vi "shear_and_recovery_integral_calculation__45bec310ce.vi"(7 "frequency":dbl, 8 "amplitude":dbl=1.0 format="%0.2f", 9 "loop period (ms)":dbl, 10 "recovery phase (half period=32)":dbl, 11 "# periods":i32) -> ()   [LabVIEW 2023]
uses:
  <vilib>/Analysis/NI_AALBase.lvlib
panel:
  out "Waveform Graph":dbl[](graph)
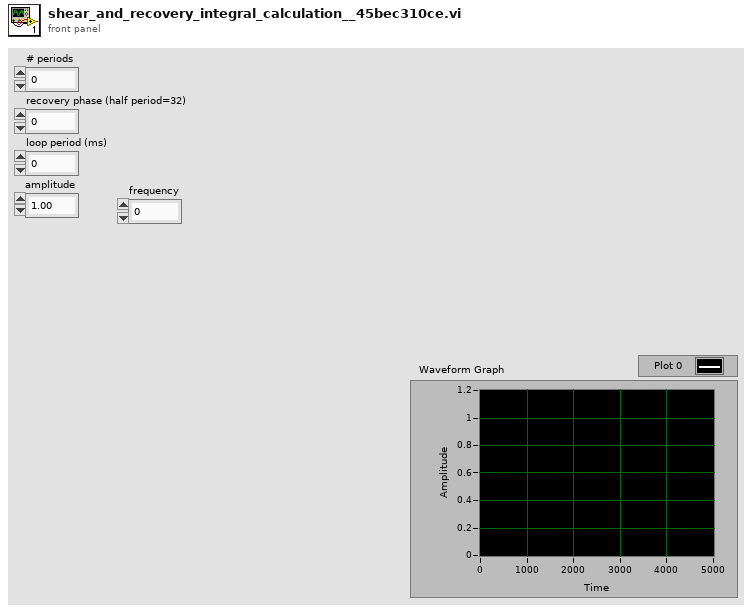
[diagram p1: front panel]
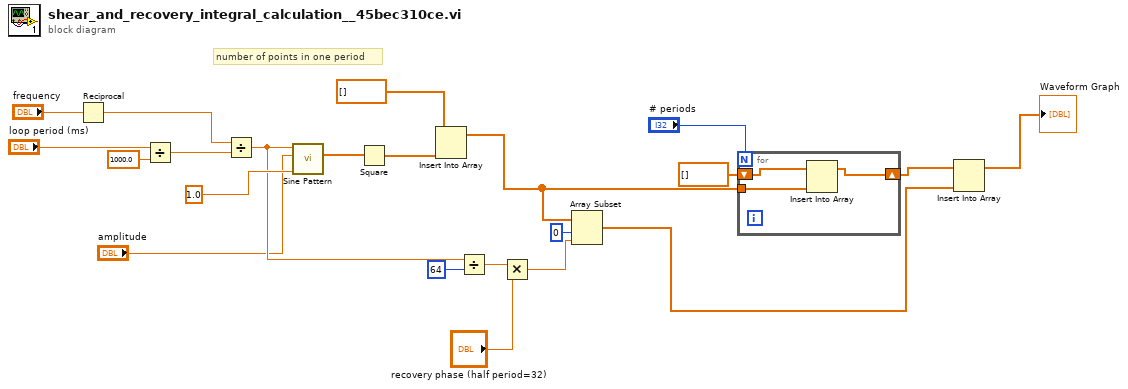
[diagram p0: block diagram]
diagram:
  # "number of points in one period"
  n1 = Reciprocal(x="frequency") -> (1/x=w8:dbl)
  n2 = Divide(x="loop period (ms)", y=1000.0) -> (x/y=w5:dbl)
  n3 = Divide(x=w8, y=w5) -> (x/y=w3:dbl)
  n4 = call <vilib>:"Sine Pattern.vi"("cycles"=1.0, "amplitude"="amplitude", "samples"=w3) -> ("Sinusoidal Pattern"=w21:dbl[])  [unwired: 1 in, 1 out]
  n5 = Square(x=w21) -> (x^2=w20:dbl[])
  n6 = Insert Into Array(array=dbl[] [], new element=w20) -> (w16:dbl[])  [unwired: 1 in]
  n7 = Divide(x=w3, y=64) -> (x/y=w14:dbl)
  n8 = Multiply(x=w14, y="recovery phase (half period=32)") -> (x*y=w11:dbl)
  n9 = Array Subset(array=w16, index=0, length=w11) -> (w10:dbl[])
  n10 = for {
    N: "# periods" -> [_]
    tunnel: w16 -> [w25]
    shift-right: [w24] -> w9
    shift-left: dbl[] [] -> [w23]
    n11 = Insert Into Array(array=w23, new element=w25) -> (w24:dbl[])  [unwired: 1 in]
  }
  n12 = Insert Into Array(array=w9, new element=w10) -> (→"Waveform Graph":dbl[])  [unwired: 1 in]
